vi "Test Select Monitored Signal B.vi"(8 "error in":errorcluster) -> (0 "error out":errorcluster)   [LabVIEW 2026]
doc: "Caraya test of Select Monitored Signal.vi: unknown IO gives valid FALSE and 0/0 (SMS-4..6)."
uses:
  <vilib>/addons/_JKI Toolkits/Caraya/classes/Test/Test.lvclass
  <vilib>/addons/_JKI Toolkits/Caraya/classes/Assert/Assert.lvclass
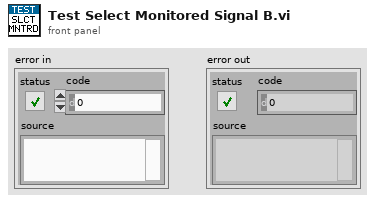
[diagram p1: front panel]
types:
  T1 = cluster{"pressure_bar":dbl, "flow_lpm":dbl, "displacement_mm":dbl, "timestamp_ms":dbl}
  T2 = cluster{"step_no":i32, "step_name":string, "command_type":string, "pressure_sp_bar":dbl, "flow_sp_lpm":dbl, "displacement_sp_mm":dbl, "monitored_io":string, "tolerance_bar":dbl, "dwell_time_ms":i32, "timeout_ms":i32, "expected_result":string}
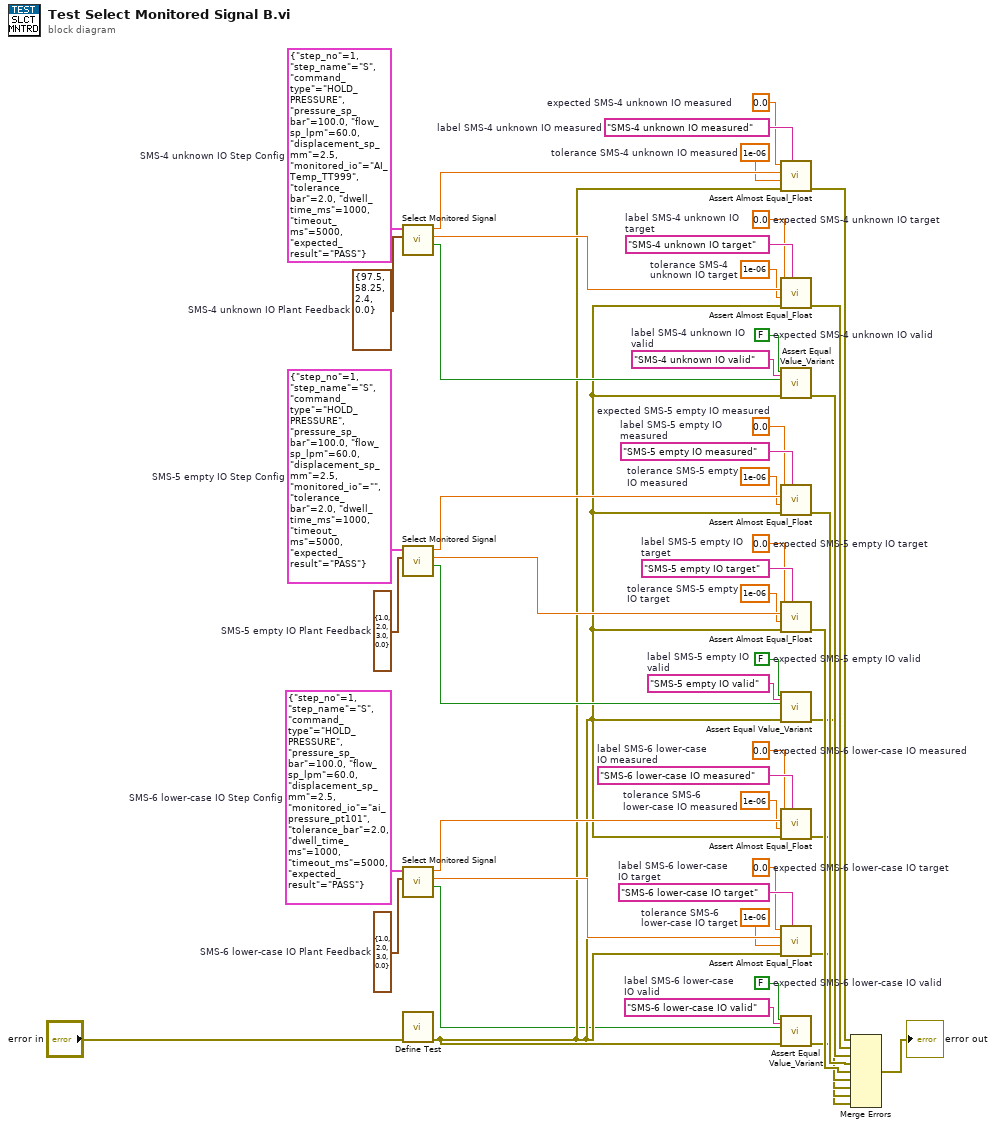
[diagram p0: block diagram]
diagram:
  w14 = "SMS-6 lower-case IO valid"  # label SMS-6 lower-case IO valid
  w12 = FALSE  # expected SMS-6 lower-case IO valid
  w18 = "SMS-6 lower-case IO target"  # label SMS-6 lower-case IO target
  w15 = 1e-06  # tolerance SMS-6 lower-case IO target
  w17 = 0.0  # expected SMS-6 lower-case IO target
  w22 = "SMS-6 lower-case IO measured"  # label SMS-6 lower-case IO measured
  w19 = 1e-06  # tolerance SMS-6 lower-case IO measured
  w21 = 0.0  # expected SMS-6 lower-case IO measured
  w23 = T1 {"pressure_bar"=1.0, "flow_lpm"=2.0, "displacement_mm"=3.0, "timestamp_ms"=0.0}  # SMS-6 lower-case IO Plant Feedback
  w24 = T2 {"step_no"=1, "step_name"="S", "command_type"="HOLD_PRESSURE", "pressure_sp_bar"=100.0, "flow_sp_lpm"=60.0, "displacement_sp_mm"=2.5, "monitored_io"="ai_pressure_pt101", "tolerance_bar"=2.0, "dwell_time_ms"=1000, "timeout_ms"=5000, "expected_result"="PASS"}  # SMS-6 lower-case IO Step Config
  w27 = "SMS-5 empty IO valid"  # label SMS-5 empty IO valid
  w26 = FALSE  # expected SMS-5 empty IO valid
  w31 = "SMS-5 empty IO target"  # label SMS-5 empty IO target
  w28 = 1e-06  # tolerance SMS-5 empty IO target
  w30 = 0.0  # expected SMS-5 empty IO target
  w35 = "SMS-5 empty IO measured"  # label SMS-5 empty IO measured
  w32 = 1e-06  # tolerance SMS-5 empty IO measured
  w34 = 0.0  # expected SMS-5 empty IO measured
  w36 = T1 {"pressure_bar"=1.0, "flow_lpm"=2.0, "displacement_mm"=3.0, "timestamp_ms"=0.0}  # SMS-5 empty IO Plant Feedback
  w37 = T2 {"step_no"=1, "step_name"="S", "command_type"="HOLD_PRESSURE", "pressure_sp_bar"=100.0, "flow_sp_lpm"=60.0, "displacement_sp_mm"=2.5, "monitored_io"="", "tolerance_bar"=2.0, "dwell_time_ms"=1000, "timeout_ms"=5000, "expected_result"="PASS"}  # SMS-5 empty IO Step Config
  w40 = "SMS-4 unknown IO valid"  # label SMS-4 unknown IO valid
  w39 = FALSE  # expected SMS-4 unknown IO valid
  w44 = "SMS-4 unknown IO target"  # label SMS-4 unknown IO target
  w41 = 1e-06  # tolerance SMS-4 unknown IO target
  w43 = 0.0  # expected SMS-4 unknown IO target
  w48 = "SMS-4 unknown IO measured"  # label SMS-4 unknown IO measured
  w45 = 1e-06  # tolerance SMS-4 unknown IO measured
  w47 = 0.0  # expected SMS-4 unknown IO measured
  w49 = T1 {"pressure_bar"=97.5, "flow_lpm"=58.25, "displacement_mm"=2.4, "timestamp_ms"=0.0}  # SMS-4 unknown IO Plant Feedback
  w50 = T2 {"step_no"=1, "step_name"="S", "command_type"="HOLD_PRESSURE", "pressure_sp_bar"=100.0, "flow_sp_lpm"=60.0, "displacement_sp_mm"=2.5, "monitored_io"="AI_Temp_TT999", "tolerance_bar"=2.0, "dwell_time_ms"=1000, "timeout_ms"=5000, "expected_result"="PASS"}  # SMS-4 unknown IO Step Config
  n1 = call "Select Monitored Signal.vi"("Plant Feedback"=w49, "Step Config"=w50) -> ("valid"=w38:bool, "target"=w42:dbl, "measured"=w46:dbl)  [unwired: 7 in]
  n2 = call "Select Monitored Signal.vi"("Plant Feedback"=w36, "Step Config"=w37) -> ("valid"=w25:bool, "target"=w29:dbl, "measured"=w33:dbl)  [unwired: 7 in]
  n3 = call "Select Monitored Signal.vi"("Plant Feedback"=w23, "Step Config"=w24) -> ("valid"=w11:bool, "target"=w16:dbl, "measured"=w20:dbl)  [unwired: 7 in]
  n4 = call <vilib>:"Define Test.vi"("error in (no error)"="error in") -> ("error out"=w13:errorcluster)  [unwired: 9 in, 1 out]
  n5 = call <vilib>:"Assert Almost Equal_Float.vi"("Label"=w48, "error in (no error)"=w13, "Tolerance"=w45, "Actual"=w46, "Expected"=w47) -> ("error out"=w10:errorcluster)  [unwired: 5 in, 1 out]
  n6 = call <vilib>:"Assert Almost Equal_Float.vi"("Label"=w44, "error in (no error)"=w13, "Tolerance"=w41, "Actual"=w42, "Expected"=w43) -> ("error out"=w9:errorcluster)  [unwired: 5 in, 1 out]
  n7 = call <vilib>:"Assert Equal Value_Variant.vi"("Label"=w40, "error in (no error)"=w13, "Actual"=w38, "Expected"=w39) -> ("error out"=w8:errorcluster)  [unwired: 6 in, 1 out]
  n8 = call <vilib>:"Assert Almost Equal_Float.vi"("Label"=w35, "error in (no error)"=w13, "Tolerance"=w32, "Actual"=w33, "Expected"=w34) -> ("error out"=w7:errorcluster)  [unwired: 5 in, 1 out]
  n9 = call <vilib>:"Assert Almost Equal_Float.vi"("Label"=w31, "error in (no error)"=w13, "Tolerance"=w28, "Actual"=w29, "Expected"=w30) -> ("error out"=w6:errorcluster)  [unwired: 5 in, 1 out]
  n10 = call <vilib>:"Assert Equal Value_Variant.vi"("Label"=w27, "error in (no error)"=w13, "Actual"=w25, "Expected"=w26) -> ("error out"=w5:errorcluster)  [unwired: 6 in, 1 out]
  n11 = call <vilib>:"Assert Almost Equal_Float.vi"("Label"=w22, "error in (no error)"=w13, "Tolerance"=w19, "Actual"=w20, "Expected"=w21) -> ("error out"=w4:errorcluster)  [unwired: 5 in, 1 out]
  n12 = call <vilib>:"Assert Almost Equal_Float.vi"("Label"=w18, "error in (no error)"=w13, "Tolerance"=w15, "Actual"=w16, "Expected"=w17) -> ("error out"=w3:errorcluster)  [unwired: 5 in, 1 out]
  n13 = call <vilib>:"Assert Equal Value_Variant.vi"("Label"=w14, "error in (no error)"=w13, "Actual"=w11, "Expected"=w12) -> ("error out"=w2:errorcluster)  [unwired: 6 in, 1 out]
  n14 = Merge Errors(w10, w9, w8, w7, w6, w5, w4, w3, w2) -> (→"error out":errorcluster)
